vi "Dialog Tester - Preempt.vi"() -> ()   [LabVIEW 2021]
doc: "<b>TEST VI</b> checking the pre-empt action for pop up types"
uses:
  src/Standard/Input (DBL)/Input (DBL).lvclass
  src/Standard/Input (I32)/Input (I32).lvclass
  src/Standard/Input (String)/Input (String).lvclass
  src/Standard/Timeout/Timeout.lvclass
  src/Standard/Timeout One Button/Timeout One Button.lvclass
  src/Standard/Timeout Two Button/Timeout Two Button.lvclass
  src/Standard/Two Button/Two Button.lvclass
  src/Popup/Popup.lvclass
panel:
  out "Two-Button T.O. Choice? - val":bool
  out "Two-Button Choice? - val":bool
  out "Input Value (String - val)":string
  out "Input Value (I32 - val)":i32
  out "Input Value (DBL - close)":dbl
  out "Two-Button T.O. Choice? - close":bool
  out "Two-Button Choice? - close":bool
  out "Input Value (String - close)":string
  out "Input Value (I32 - close)":i32
  out "Input Value (DBL - val)":dbl
  out "iteration":i32
  in  "Error In":errorcluster
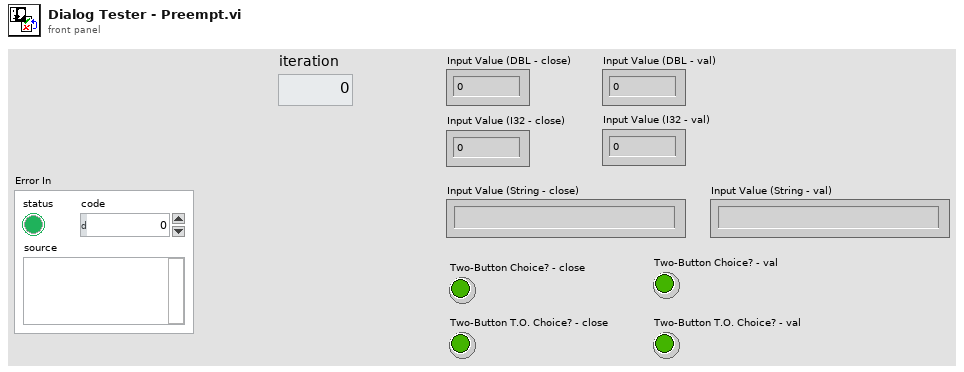
[diagram p1: front panel]
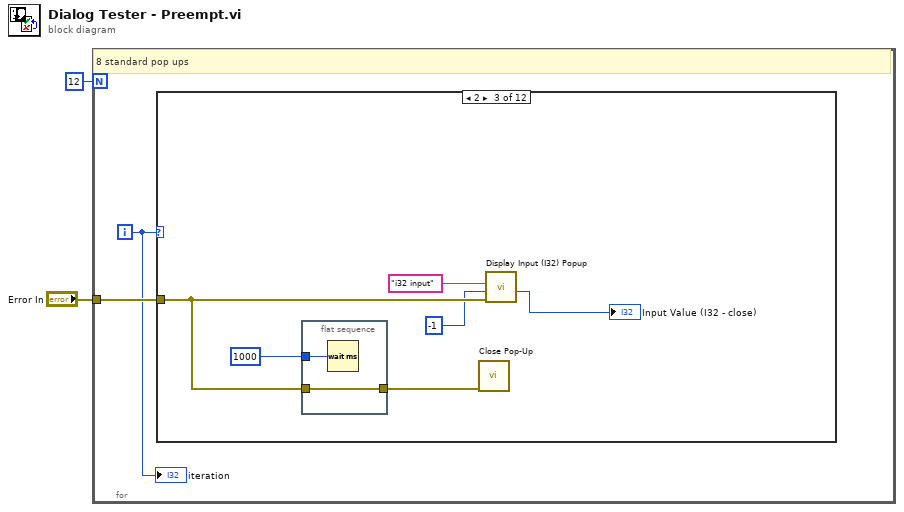
[diagram p0: block diagram]
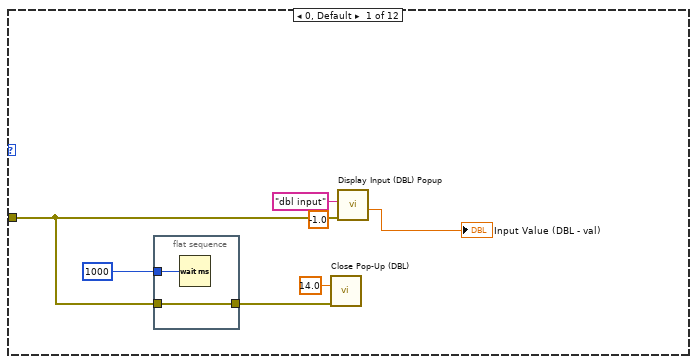
[diagram p2: hidden frame]
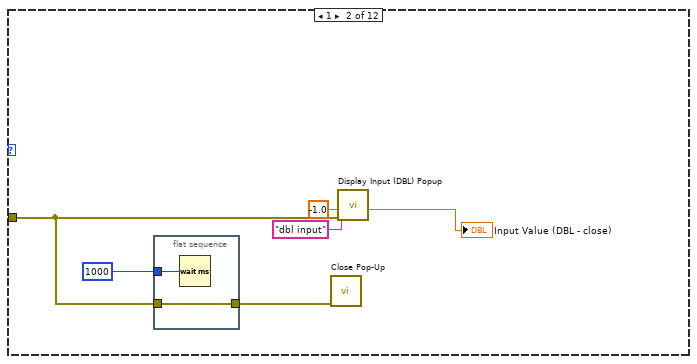
[diagram p3: hidden frame]
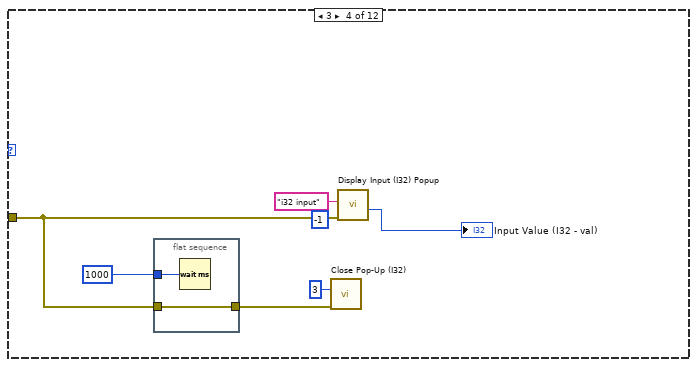
[diagram p4: hidden frame]
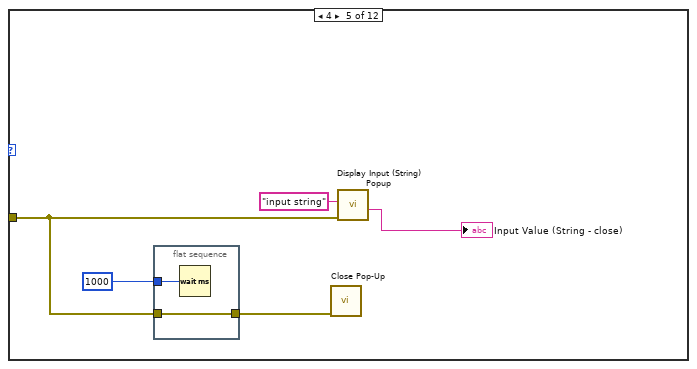
[diagram p5: hidden frame]
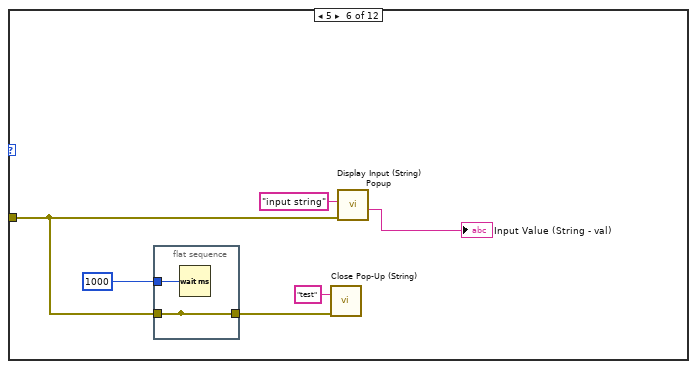
[diagram p6: hidden frame]
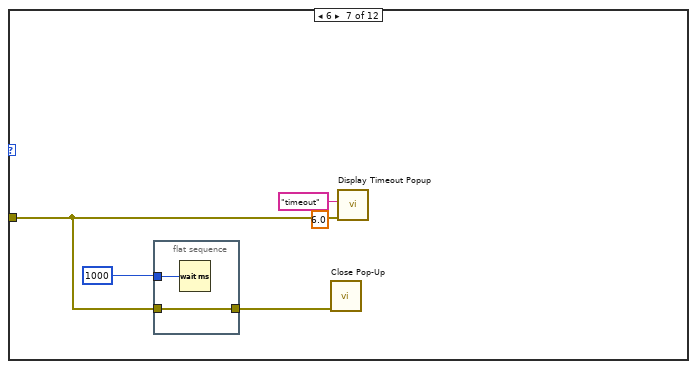
[diagram p7: hidden frame]
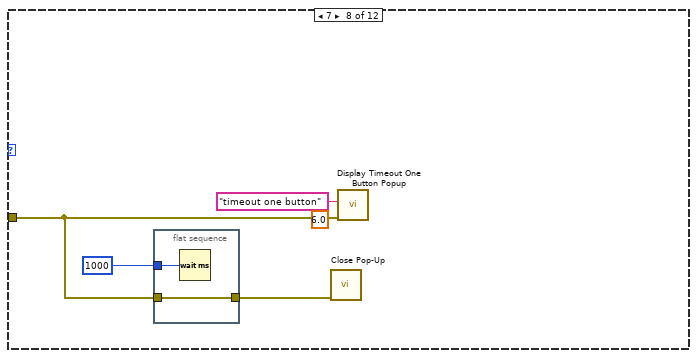
[diagram p8: hidden frame]
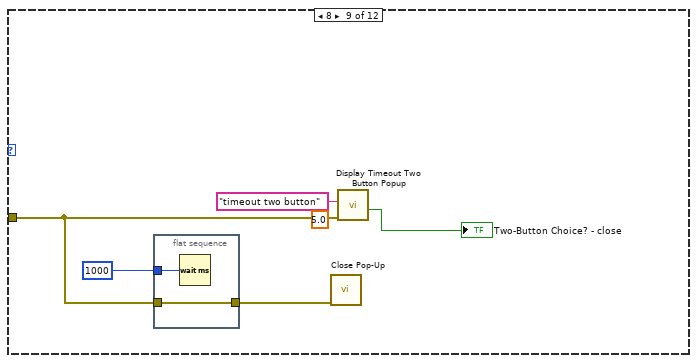
[diagram p9: hidden frame]
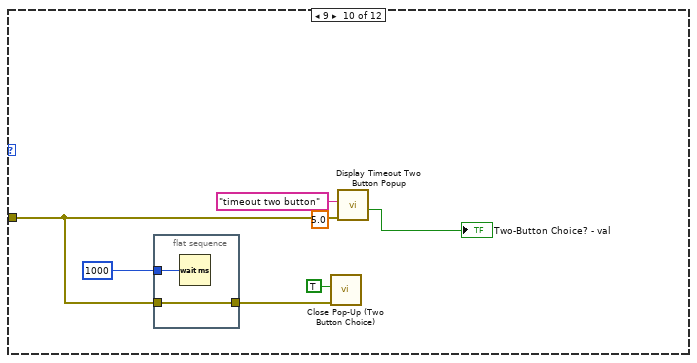
[diagram p10: hidden frame]
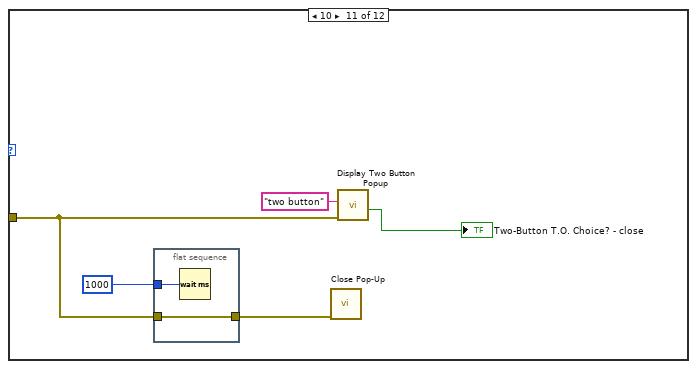
[diagram p11: hidden frame]
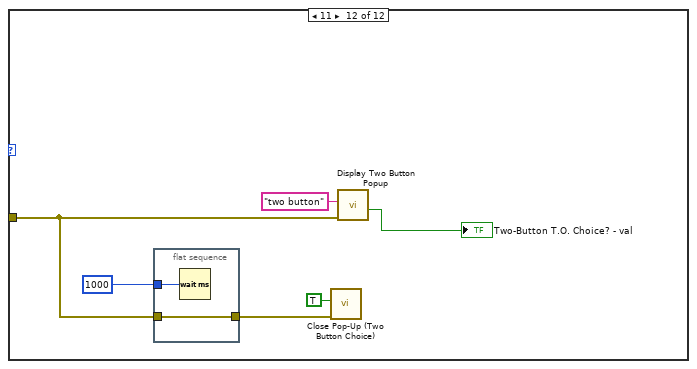
[diagram p12: hidden frame]
diagram:
  n1 = for {
    N: 12 -> [_]
    tunnel: "Error In" -> [w4]
    i -> [w3]
    # "8 standard pop ups"
    n2 = case shown="2" w3 {
      tunnel: w4 -> [w11 w19 w26 w35 w42 w50 w56 w64 w72 w81 w88 w96]
      frame 0, Default {
        n3 = flat-sequence {
          tunnel: u32 1000 ("milliseconds to wait") -> [w12]
          tunnel: [w13] -> w10
          tunnel: w11 -> [w13]
          frame #0 {
            n4 = Wait (ms)(milliseconds to wait=w12) -> ()  [unwired: 1 out]
          }
        }
        n5 = call "Close Pop-Up (DBL).vi"("error in"=w10, "DBL Default"=14.0) -> ()  [unwired: 9 in, 1 out]
        n6 = call "Display Input (DBL) Popup.vi"("error in"=w11, "Default Input"=-1.0, "Message"="dbl input") -> ("Input Value"=→"Input Value (DBL - val)":dbl)  [unwired: 7 in, 1 out]
      }
      frame 1 {
        n7 = flat-sequence {
          tunnel: u32 1000 ("milliseconds to wait") -> [w20]
          tunnel: [w21] -> w18
          tunnel: w19 -> [w21]
          frame #0 {
            n8 = Wait (ms)(milliseconds to wait=w20) -> ()  [unwired: 1 out]
          }
        }
        n9 = call "Close Pop-Up.vi"("error in"=w18) -> ()  [unwired: 10 in, 1 out]
        n10 = call "Display Input (DBL) Popup.vi"("error in"=w19, "Default Input"=-1.0, "Message"="dbl input") -> ("Input Value"=→"Input Value (DBL - close)":dbl)  [unwired: 7 in, 1 out]
      }
      frame 2 {
        n11 = flat-sequence {
          tunnel: u32 1000 ("milliseconds to wait") -> [w28]
          tunnel: [w29] -> w27
          tunnel: w26 -> [w29]
          frame #0 {
            n12 = Wait (ms)(milliseconds to wait=w28) -> ()  [unwired: 1 out]
          }
        }
        n13 = call "Close Pop-Up.vi"("error in"=w27) -> ()  [unwired: 10 in, 1 out]
        n14 = call "Display Input (I32) Popup.vi"("error in"=w26, "Default Input"=-1, "Message"="i32 input") -> ("Input Value"=→"Input Value (I32 - close)":i32)  [unwired: 7 in, 1 out]
      }
      frame 3 {
        n15 = flat-sequence {
          tunnel: u32 1000 ("milliseconds to wait") -> [w36]
          tunnel: [w37] -> _
          tunnel: w35 -> [w37]
          frame #0 {
            n16 = Wait (ms)(milliseconds to wait=w36) -> ()  [unwired: 1 out]
          }
        }
        n17 = call "Close Pop-Up (I32).vi"("error in"=w35, "I32 Default"=3) -> ()  [unwired: 9 in, 1 out]
        n18 = call "Display Input (I32) Popup.vi"("error in"=w35, "Default Input"=-1, "Message"="i32 input") -> ("Input Value"=→"Input Value (I32 - val)":i32)  [unwired: 7 in, 1 out]
      }
      frame 4 {
        n19 = flat-sequence {
          tunnel: u32 1000 ("milliseconds to wait") -> [w43]
          tunnel: [w44] -> w41
          tunnel: w42 -> [w44]
          frame #0 {
            n20 = Wait (ms)(milliseconds to wait=w43) -> ()  [unwired: 1 out]
          }
        }
        n21 = call "Close Pop-Up.vi"("error in"=w41) -> ()  [unwired: 10 in, 1 out]
        n22 = call "Display Input (String) Popup.vi"("error in"=w42, "Message"="input string") -> ("Input Value"=→"Input Value (String - close)":string)  [unwired: 8 in, 1 out]
      }
      frame 5 {
        n23 = flat-sequence {
          tunnel: u32 1000 ("milliseconds to wait") -> [w51]
          tunnel: [w52] -> w49
          tunnel: [w52] -> _
          tunnel: w50 -> [w52]
          frame #0 {
            n24 = Wait (ms)(milliseconds to wait=w51) -> ()  [unwired: 1 out]
          }
        }
        n25 = call "Close Pop-Up (String).vi"("error in"=w49, "String Default"="test") -> ()  [unwired: 9 in, 1 out]
        n26 = call "Display Input (String) Popup.vi"("error in"=w50, "Message"="input string") -> ("Input Value"=→"Input Value (String - val)":string)  [unwired: 8 in, 1 out]
      }
      frame 6 {
        n27 = flat-sequence {
          tunnel: u32 1000 ("milliseconds to wait") -> [w58]
          tunnel: [w59] -> w57
          tunnel: w56 -> [w59]
          frame #0 {
            n28 = Wait (ms)(milliseconds to wait=w58) -> ()  [unwired: 1 out]
          }
        }
        n29 = call "Close Pop-Up.vi"("error in"=w57) -> ()  [unwired: 10 in, 1 out]
        n30 = call "Display Timeout Popup.vi"("error in"=w56, "Timeout (s)"=6.0, "Message"="timeout") -> ()  [unwired: 7 in, 2 out]
      }
      frame 7 {
        n31 = flat-sequence {
          tunnel: u32 1000 ("milliseconds to wait") -> [w65]
          tunnel: [w66] -> w63
          tunnel: w64 -> [w66]
          frame #0 {
            n32 = Wait (ms)(milliseconds to wait=w65) -> ()  [unwired: 1 out]
          }
        }
        n33 = call "Close Pop-Up.vi"("error in"=w63) -> ()  [unwired: 10 in, 1 out]
        n34 = call "Display Timeout One Button Popup.vi"("error in"=w64, "Timeout (s)"=6.0, "Message"="timeout one button") -> ()  [unwired: 7 in, 2 out]
      }
      frame 8 {
        n35 = flat-sequence {
          tunnel: u32 1000 ("milliseconds to wait") -> [w73]
          tunnel: [w74] -> w71
          tunnel: w72 -> [w74]
          frame #0 {
            n36 = Wait (ms)(milliseconds to wait=w73) -> ()  [unwired: 1 out]
          }
        }
        n37 = call "Close Pop-Up.vi"("error in"=w71) -> ()  [unwired: 10 in, 1 out]
        n38 = call "Display Timeout Two Button Popup.vi"("error in"=w72, "Timeout (s)"=5.0, "Message"="timeout two button") -> ("Choice"=→"Two-Button Choice? - close":bool)  [unwired: 6 in, 2 out]
      }
      frame 9 {
        n39 = flat-sequence {
          tunnel: u32 1000 ("milliseconds to wait") -> [w82]
          tunnel: [w83] -> w80
          tunnel: w81 -> [w83]
          frame #0 {
            n40 = Wait (ms)(milliseconds to wait=w82) -> ()  [unwired: 1 out]
          }
        }
        n41 = call "Close Pop-Up (Two Button Choice).vi"("error in"=w80, "Two-Button Choice? (F)"=TRUE) -> ()  [unwired: 9 in, 1 out]
        n42 = call "Display Timeout Two Button Popup.vi"("error in"=w81, "Timeout (s)"=5.0, "Message"="timeout two button") -> ("Choice"=→"Two-Button Choice? - val":bool)  [unwired: 6 in, 2 out]
      }
      frame 10 {
        n43 = flat-sequence {
          tunnel: u32 1000 ("milliseconds to wait") -> [w89]
          tunnel: [w90] -> w87
          tunnel: w88 -> [w90]
          frame #0 {
            n44 = Wait (ms)(milliseconds to wait=w89) -> ()  [unwired: 1 out]
          }
        }
        n45 = call "Close Pop-Up.vi"("error in"=w87) -> ()  [unwired: 10 in, 1 out]
        n46 = call "Display Two Button Popup.vi"("error in"=w88, "Message"="two button") -> ("Choice"=→"Two-Button T.O. Choice? - close":bool)  [unwired: 8 in, 1 out]
      }
      frame 11 {
        n47 = flat-sequence {
          tunnel: u32 1000 ("milliseconds to wait") -> [w97]
          tunnel: [w98] -> w95
          tunnel: w96 -> [w98]
          frame #0 {
            n48 = Wait (ms)(milliseconds to wait=w97) -> ()  [unwired: 1 out]
          }
        }
        n49 = call "Close Pop-Up (Two Button Choice).vi"("error in"=w95, "Two-Button Choice? (F)"=TRUE) -> ()  [unwired: 9 in, 1 out]
        n50 = call "Display Two Button Popup.vi"("error in"=w96, "Message"="two button") -> ("Choice"=→"Two-Button T.O. Choice? - val":bool)  [unwired: 8 in, 1 out]
      }
    }
    "iteration" <- w3
  }
